vi "DSS-Tests-run_all.vi"() -> ()   [LabVIEW 2020, in "DSS-Tests.lvlib"]
doc: "Runs every DSS Caraya test VI of this folder (paths relative to this VI) non-interactively and writes the JUnit report DSS-Tests-run_all-TestReport.xml beside it."
uses:
  DSS-Tests.lvlib
  <vilib>/addons/_JKI Toolkits/Caraya/Caraya.lvlib
panel:
  out "error out":errorcluster
  out "Report Path used":path
  in  "error in":errorcluster
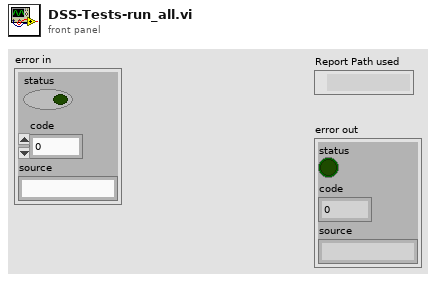
[diagram p1: front panel]
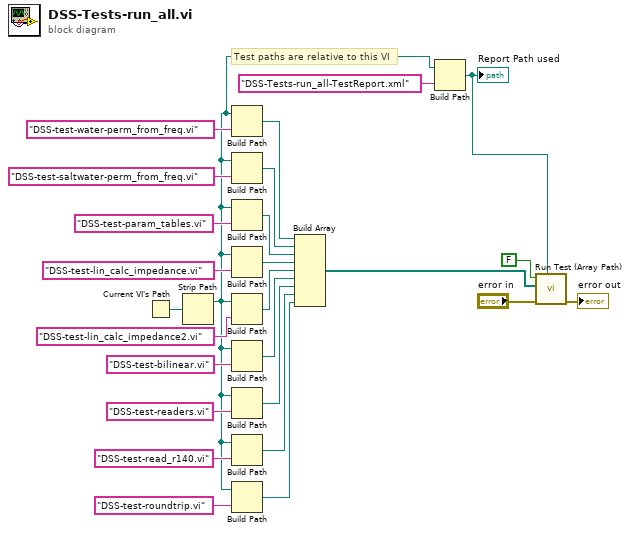
[diagram p0: block diagram]
diagram:
  # "Test paths are relative to this VI"
  n1 = Current VI's Path() -> (path=w1:path)
  n2 = Strip Path(path=w1) -> (stripped path=w2:path)  [unwired: 1 out]
  n3 = Build Path(base path=w2, name or relative path="DSS-test-water-perm_from_freq.vi" ("name or relative path 1")) -> (appended path=w13:path)
  n4 = Build Path(base path=w2, name or relative path="DSS-test-saltwater-perm_from_freq.vi" ("name or relative path 2")) -> (appended path=w14:path)
  n5 = Build Path(base path=w2, name or relative path="DSS-test-param_tables.vi" ("name or relative path 3")) -> (appended path=w15:path)
  n6 = Build Path(base path=w2, name or relative path="DSS-test-lin_calc_impedance.vi" ("name or relative path 4")) -> (appended path=w16:path)
  n7 = Build Path(base path=w2, name or relative path="DSS-test-lin_calc_impedance2.vi" ("name or relative path 5")) -> (appended path=w17:path)
  n8 = Build Path(base path=w2, name or relative path="DSS-test-bilinear.vi" ("name or relative path 6")) -> (appended path=w18:path)
  n9 = Build Path(base path=w2, name or relative path="DSS-test-readers.vi" ("name or relative path 7")) -> (appended path=w19:path)
  n10 = Build Path(base path=w2, name or relative path="DSS-test-read_r140.vi" ("name or relative path 8")) -> (appended path=w20:path)
  n11 = Build Path(base path=w2, name or relative path="DSS-test-roundtrip.vi" ("name or relative path 9")) -> (appended path=w21:path)
  n12 = Build Array(w13, w14, w15, w16, w17, w18, w19, w20, w21) -> (w23:path[])
  n13 = Build Path(base path=w2, name or relative path="DSS-Tests-run_all-TestReport.xml" ("report file name")) -> (appended path=w22:path)
  "Report Path used" <- w22
  n14 = call <vilib>:"Run Test (Array Path).vi"("Report Path"=w22, "error in"="error in", "Paths"=w23, "Interactive (T)"=FALSE) -> ("error out"=→"error out":errorcluster)  [unwired: 6 in, 1 out]
